vi "test.vi"() -> ()   [LabVIEW 2018]
uses:
  Content/TypeDef/EventTypeDef.ctl
  <vilib>/httpClient/POSTBuffer.vi
  HASS-LV-WS_integration.lvlib
  <vilib>/MediaMongrels Ltd/WebSockets/WebSockets/WebSockets.lvlib
  <vilib>/httpClient/LabVIEWHTTPClient.lvlib
panel:
  in  "Tab Control":T1(tab)
  out "Connection Result":string
  out "Connection Authenticated?":bool
  out "Event Data (WS)":string
  in  "Call Service Data":T2
  out "Event Name (WS)":string
  in  "Event":string
  in  "Add Button":bool
  in  "Remove Button":bool
  in  "call service btn":bool
  out "States (WS)":T3(array[cluster])
  in  "Fetch states":bool
  out "Success":bool
  out "States (REST)":T3(array[cluster])
  in  "Fetch states REST":bool
  out "State":T4
  in  "Fetch state REST":bool
  in  "entity_name":string="sun.sun"
  out "Base URL":string="sun.sun"
  in  "HTTP GET":bool
  out "HTTP GET RESPONSE":string
  in  "GET URL":string="sun.sun"
  in  "HTTP POST":bool
  out "HTTP POST RESPONSE":string
  in  "POST URL":string
  in  "Text To Send":string
  out "Base URL 2":string="sun.sun" caption="Base URL"
  in  "Stop Button":bool
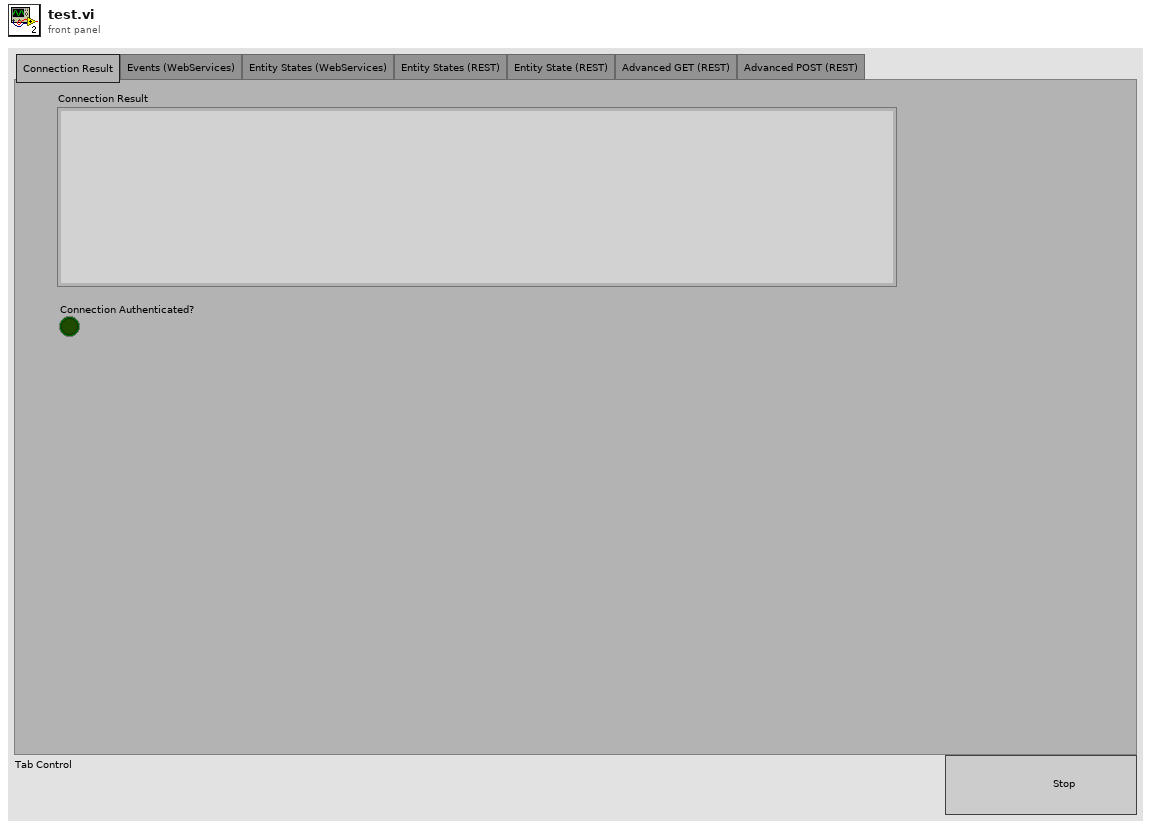
[diagram p1: front panel]
types:
  T1 = enum32{"Connection Result", "Events (WebServices)", "Entity States (WebServices)", "Entity States (REST)", "Entity State (REST)", "Advanced GET (REST)", "Advanced POST (REST)"}
  T2 = cluster{"Service Domain":string, "Service":string, "Optional - Service Data (JSON string)":string}
  T3 = cluster{"entity_id":string, "state":string, "last_changed":string, "last_updated":string, "attributes":cluster{"key":string, "value":string}[], "context":cluster{"key":string, "value":string}[]}[]
  T4 = cluster{"entity_id":string, "state":string, "last_changed":string, "last_updated":string, "attributes":cluster{"key":string, "value":string}[], "context":cluster{"key":string, "value":string}[]}
  T5 = typedef "HASS-LV-WS_integration.lvlib/ReferencesTypeDef.ctl" = cluster{"user event":refnum<user-event>, "send queue":refnum<queue>, "receive queue":refnum<queue>, "TCP Network Connection":refnum<k5>, "ws engine notifier ":refnum<notifier>, "Event Registration Refnum":refnum<event-registration>}
  T6 = typedef "LabVIEWHTTPClient.lvlib/ClientHandle.ctl" = refnum<k1>
  T7 = typedef "HASS-LV-WS_integration.lvlib/EventTypeDef.ctl" = cluster{"Data":variant, "Command":string}
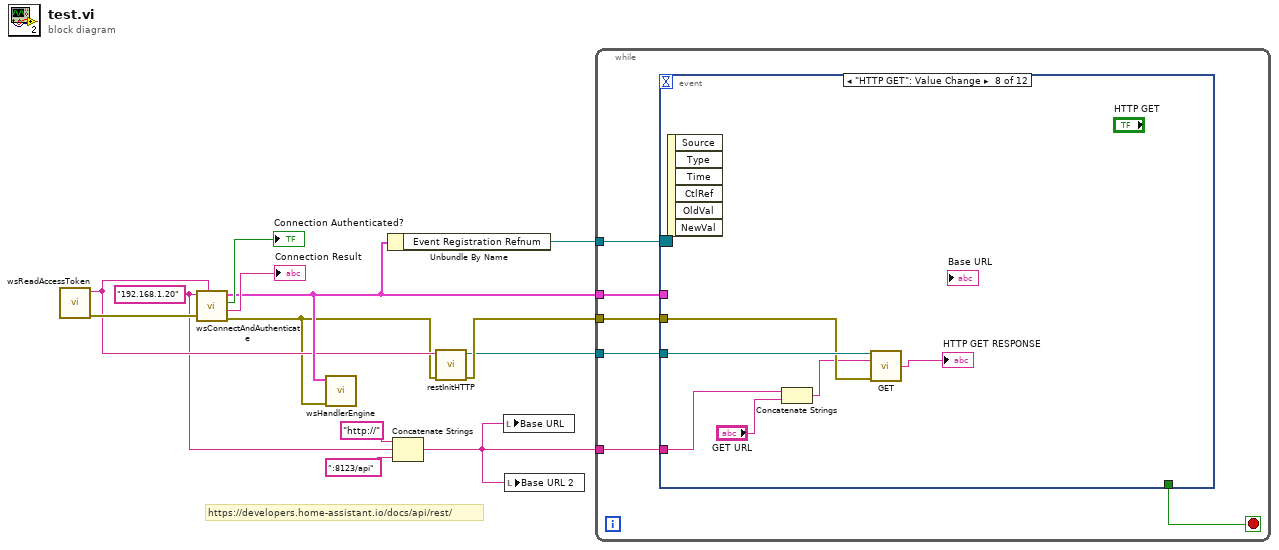
[diagram p0: block diagram]
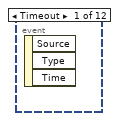
[diagram p2: hidden frame]
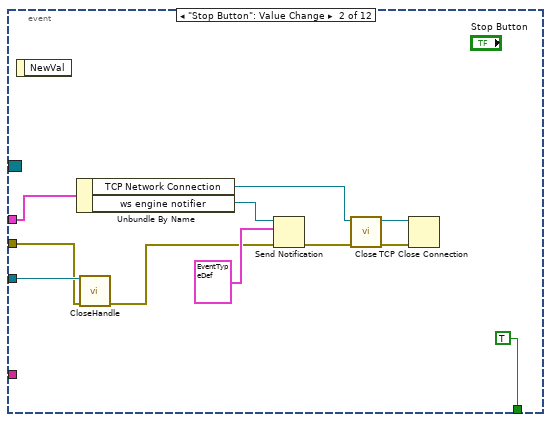
[diagram p3: hidden frame]
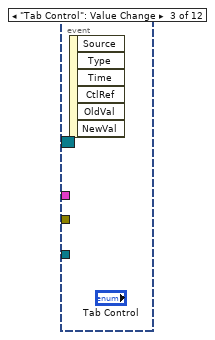
[diagram p4: hidden frame]
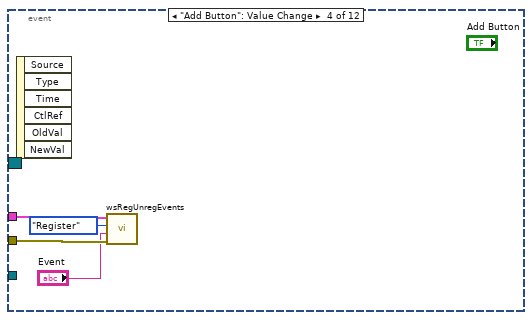
[diagram p5: hidden frame]
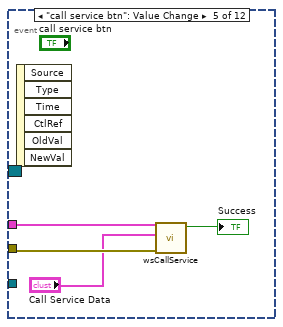
[diagram p6: hidden frame]
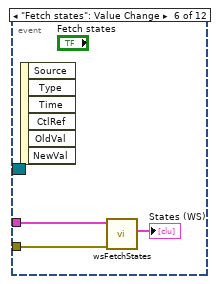
[diagram p7: hidden frame]
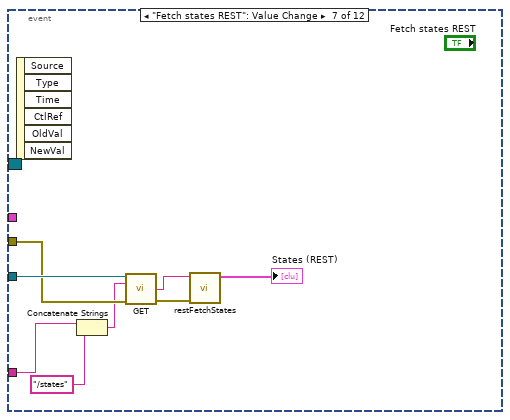
[diagram p8: hidden frame]
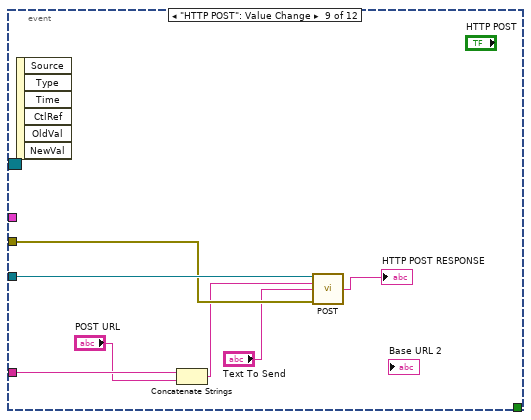
[diagram p9: hidden frame]
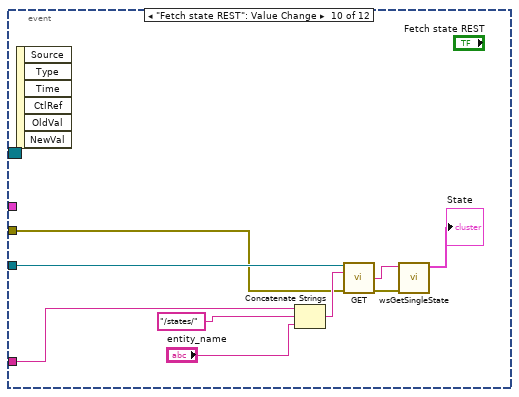
[diagram p10: hidden frame]
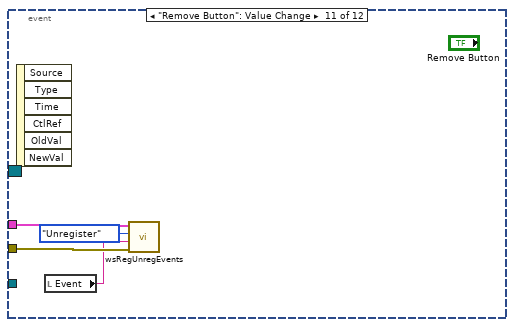
[diagram p11: hidden frame]
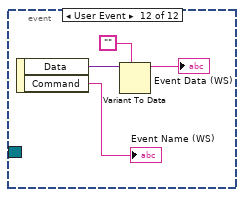
[diagram p12: hidden frame]
diagram:
  w3 = "192.168.1.20" ("Server Address")
  # "https://developers.home-assistant.io/docs/api/rest/"
  n1 = call "wsReadAccessToken.vi"() -> ("error out"=w9:errorcluster, "access token"=w8:string)  [unwired: 9 in, 1 out]
  n2 = call "wsConnectAndAuthenticate.vi"("Access Token"=w8, "error in (no error)"=w9, "Server Address"=w3) -> ("error out"=w7:errorcluster, "Connection Result"=→"Connection Result":string, "Connection Authenticated?"=→"Connection Authenticated?":bool, "References"=w10:T5)  [unwired: 5 in]
  n3 = call "wsHandlerEngine.vi"("error in (no error)"=w7, "References"=w10) -> ()  [unwired: 9 in, 1 out]
  n4 = Unbundle By Name(w10) -> ("Event Registration Refnum"=w11:refnum<event-registration>)
  n5 = Concatenate Strings("http://" ("string"), w3, ":8123/api" ("string")) -> (w1:string)
  n6 = call "restInitHTTP.vi"("error in (no error)"=w7, "access token"=w8) -> ("error out"=w6:errorcluster, "Refnum out"=w5:T6)  [unwired: 8 in]
  n7 = local write "Base URL"(w1) -> ()
  n8 = local write "Base URL 2"(w1) -> ()
  n9 = while {
    tunnel: w10 -> [w18]
    tunnel: w6 -> [w17]
    tunnel: w11 -> [w16]
    tunnel: w5 -> [w15]
    tunnel: w1 -> [w14]
    stop <- w19 stop-if-true
    n10 = event shown="[7] \"HTTP GET\": Value Change" {
      selector: w16 -> [_ _ _ _ _ _ _ _ _ _ _ _]
      dyn-events: _ -> [_ _ _ _ _ _ _ _ _ _ _ _]
      timeout: _ -> [_ _ _ _ _ _ _ _ _ _ _ _]
      tunnel: [_ TRUE _ _ _ _ _ _ _ _ _ _] -> w19
      tunnel: w18 -> [_ w29 _ w34 w37 w40 _ _ _ _ w74 _]
      tunnel: w17 -> [_ w21 _ w33 w38 w41 w48 w54 w60 w66 w75 _]
      tunnel: w15 -> [_ w22 _ _ _ _ w49 w55 w62 w70 _ _]
      tunnel: w14 -> [_ _ _ _ _ _ w47 w53 w58 w65 _ _]
      event Timeout {
        n11 = event-data() -> ()  [unwired: 1 in, 3 out]
      }
      event "Stop Button": Value Change {
        n12 = event-data() -> ()  [unwired: 1 in, 1 out]
        n13 = Unbundle By Name(w29) -> ("TCP Network Connection"=w25:refnum<k5>, "ws engine notifier"=w28:refnum<notifier>)
        n14 = call <vilib>:"CloseHandle.vi"("client handle"=w22, "error in (no error)"=w21) -> ("error out"=w20:errorcluster)  [unwired: 13 in]
        n15 = Send Notification(notification=T7 {"Data"=variant, "Command"="Quit"}, notifier=w28, error in (no error)=w20) -> (error out=w27:errorcluster)  [unwired: 1 out]
        n16 = call <vilib>:"Close.vi"("error in (no error)"=w27, "WebSocket Connection in"=w25) -> ("error out"=w26:errorcluster, "WebSocket Connection in"=w24:refnum<k5>)  [unwired: 8 in]
        n17 = TCP Close Connection(connection ID=w24, error in (no error)=w26) -> ()  [unwired: 1 in, 2 out]
      }
      event "Tab Control": Value Change {
        n18 = event-data() -> ()  [unwired: 1 in, 6 out]
      }
      event "Add Button": Value Change {
        n19 = event-data() -> ()  [unwired: 1 in, 6 out]
        n20 = call "wsRegUnregEvents.vi"("Error In"=w33, "Event Name (empty =all)"="Event", "Action"=enum16{"Register", "Unregister"}."Register", "References"=w34) -> ()  [unwired: 7 in, 1 out]
      }
      event "call service btn": Value Change {
        n21 = event-data() -> ()  [unwired: 1 in, 6 out]
        n22 = call "wsCallService.vi"("error in (no error)"=w38, "Call Service Data"="Call Service Data", "References"=w37) -> ("Success?"=→"Success":bool)  [unwired: 7 in, 1 out]
      }
      event "Fetch states": Value Change {
        n23 = event-data() -> ()  [unwired: 1 in, 6 out]
        n24 = call "wsFetchStates.vi"("error in (no error)"=w41, "References"=w40) -> ("states"=→"States (WS)":T3)  [unwired: 7 in, 2 out]
      }
      event "Fetch states REST": Value Change {
        n25 = event-data() -> ()  [unwired: 1 in, 6 out]
        n26 = Concatenate Strings(w47, "/states" ("url")) -> (w45:string)
        n27 = call <vilib>:"GET.vi"("client handle"=w49, "url"=w45, "error in (no error)"=w48) -> ("body"=w44:string, "error out"=w43:errorcluster)  [unwired: 9 in, 2 out]
        n28 = call "restFetchStates.vi"("error in (no error)"=w43, "JSON String"=w44) -> ("states"=→"States (REST)":T3)  [unwired: 8 in, 1 out]
      }
      event "HTTP GET": Value Change {
        n29 = event-data() -> ()  [unwired: 1 in, 6 out]
        n30 = Concatenate Strings(w53, "GET URL") -> (w52:string)
        n31 = call <vilib>:"GET.vi"("client handle"=w55, "url"=w52, "error in (no error)"=w54) -> ("body"=→"HTTP GET RESPONSE":string)  [unwired: 9 in, 3 out]
      }
      event "HTTP POST": Value Change {
        n32 = event-data() -> ()  [unwired: 1 in, 6 out]
        n33 = Concatenate Strings(w58, "POST URL") -> (w57:string)
        n34 = call-poly <vilib>:"POST.vi"("client handle"=w62, "url"=w57, "buffer"="Text To Send", "error in (no error)"=w60) -> ("body"=→"HTTP POST RESPONSE":string)  [unwired: 8 in, 3 out]
      }
      event "Fetch state REST": Value Change {
        n35 = event-data() -> ()  [unwired: 1 in, 6 out]
        n36 = Concatenate Strings(w65, "/states/" ("url"), "entity_name") -> (w71:string)
        n37 = call <vilib>:"GET.vi"("client handle"=w70, "url"=w71, "error in (no error)"=w66) -> ("body"=w68:string, "error out"=w67:errorcluster)  [unwired: 9 in, 2 out]
        n38 = call "wsGetSingleState.vi"("error in (no error)"=w67, "JSON String"=w68) -> ("State"=→"State":T4)  [unwired: 8 in, 1 out]
      }
      event "Remove Button": Value Change {
        n39 = event-data() -> ()  [unwired: 1 in, 6 out]
        n40 = local read "Event"() -> (w73:string)
        n41 = call "wsRegUnregEvents.vi"("Error In"=w75, "Event Name (empty =all)"=w73, "Action"=enum16{"Register", "Unregister"}."Unregister", "References"=w74) -> ()  [unwired: 7 in, 1 out]
      }
      event User Event {
        n42 = event-data() -> ("Data"=w78:variant, "Command"=→"Event Name (WS)":string)  [unwired: 1 in]
        n43 = Variant To Data(type="", Variant=w78) -> (data=→"Event Data (WS)":string)  [unwired: 1 in, 1 out]
      }
    }
  }
